vi "ms_LLSE.vi"(4 "error in (no error)":errorcluster, 5 "b":cdb[](array[numeric]), 7 "A":cdb[][](array[numeric]) format="%0.2f") -> (0 "error out":errorcluster, 2 "mean square error":dbl, 3 "x.estimate":cdb[](array[numeric]))   [LabVIEW 2026]
uses:
  <vilib>/Analysis/baseanly.llb/Complex A x B.vi
  <vilib>/Analysis/baseanly.llb/Complex A x Vector.vi
  <vilib>/Analysis/baseanly.llb/Complex Vector x A.vi
  <vilib>/Analysis/baseanly.llb/Complex Inverse Matrix.vi
  <vilib>/Analysis/NI_AALBase.lvlib
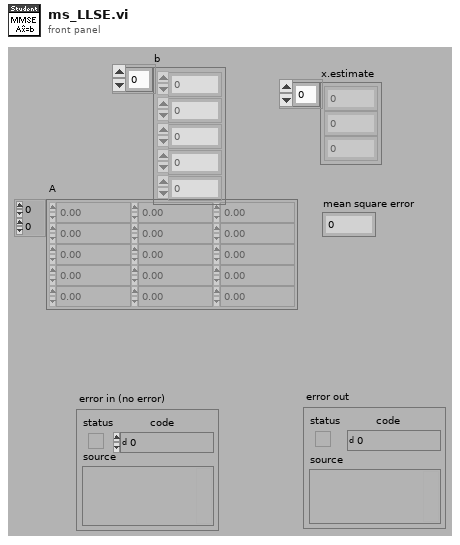
[diagram p1: front panel]
types:
  T1 = typedef "NI_Matrix.lvlib/ComplexMatrix.ctl" = cdb[][]
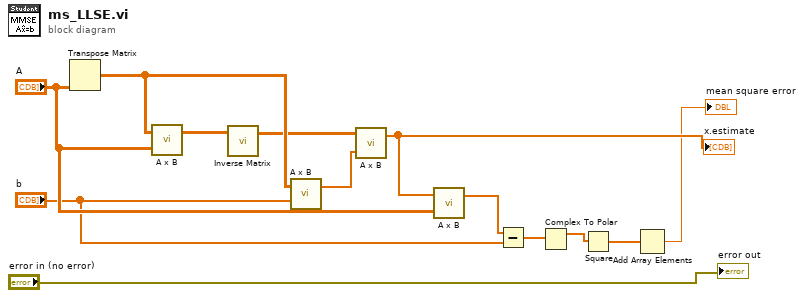
[diagram p0: block diagram]
diagram:
  n1 = Transpose Matrix(1:"A") -> (0:w12:cdb[][])
  n2 = call-poly <vilib>:"A x B.vi"("B"="A", "A"=w12) -> ("A x B"=w13:T1)  [unwired: 1 out]
  n3 = call-poly <vilib>:"Inverse Matrix.vi"("Input Matrix"=w13) -> ("Inverse Matrix"=w11:T1)  [unwired: 1 in, 1 out]
  n4 = call-poly <vilib>:"A x B.vi"("Vector"="b", "A"=w12) -> ("A x Vector"=w10:cdb[])  [unwired: 1 out]
  n5 = call-poly <vilib>:"A x B.vi"("Vector"=w10, "A"=w11) -> ("A x Vector"=w8:cdb[])  [unwired: 1 out]
  "x.estimate" <- w8
  n6 = call-poly <vilib>:"A x B.vi"("Matrix A"="A", "Vector V'"=w8) -> ("V' x A"=w7:cdb[])  [unwired: 1 out]
  n7 = Subtract(x=w7, y="b") -> (x-y=w5:cdb[])
  n8 = Complex To Polar(r * e^(i*theta)=w5) -> (r=w4:dbl[])  [unwired: 1 out]
  n9 = Square(x=w4) -> (x^2=w3:dbl[])
  n10 = Add Array Elements(numeric array=w3) -> (sum=→"mean square error":dbl)
  "error out" <- "error in (no error)"
